vi "OwnMergeObjectOwner.vi"() -> ()   [LabVIEW 2024]
panel:
  out "error out":errorcluster caption="错误输出"
  out "owner_id":refnum<vi>
  in  "object_id":u32
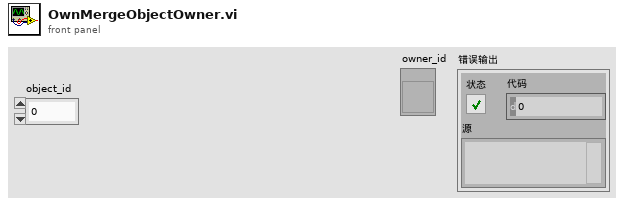
[diagram p1: front panel]
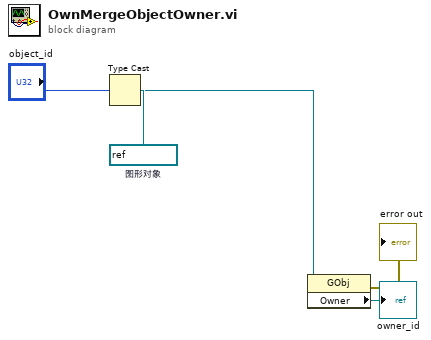
[diagram p0: block diagram]
diagram:
  w4 = refnum<vi> refnum  # 图形对象
  n1 = Type Cast ("强制类型转换")(type=w4, x="object_id") -> (*(type *) &x=w1:refnum<vi>)
  n2 = property on="属性节点" class="GObj"(reference=w1) -> (error out=→"error out":errorcluster, "Owner"=→"owner_id":refnum<vi>)  [unwired: 1 in, 1 out]
